vi "lire config gene.vi"(2 "error in":errorcluster, 3 "refnum":T1) -> (0 "error out":errorcluster, 1 "refnum out":T1)   [LabVIEW 2022 SP3]
uses:
  <vilib>/Utility/config.llb/Config Data RefNum.ctl
  <vilib>/Utility/config.llb/Read Key (Path).vi
  Variables globales/Variable glob generale.vi
  <vilib>/Utility/config.llb/Read Key (String).vi
  Variables globales/Variable glob mails.vi
  <vilib>/Utility/config.llb/NI_LVConfig.lvlib
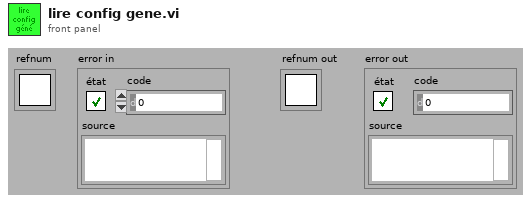
[diagram p1: front panel]
types:
  T1 = typedef "NI_LVConfig.lvlib/Config Data RefNum.ctl" = refnum<k1>
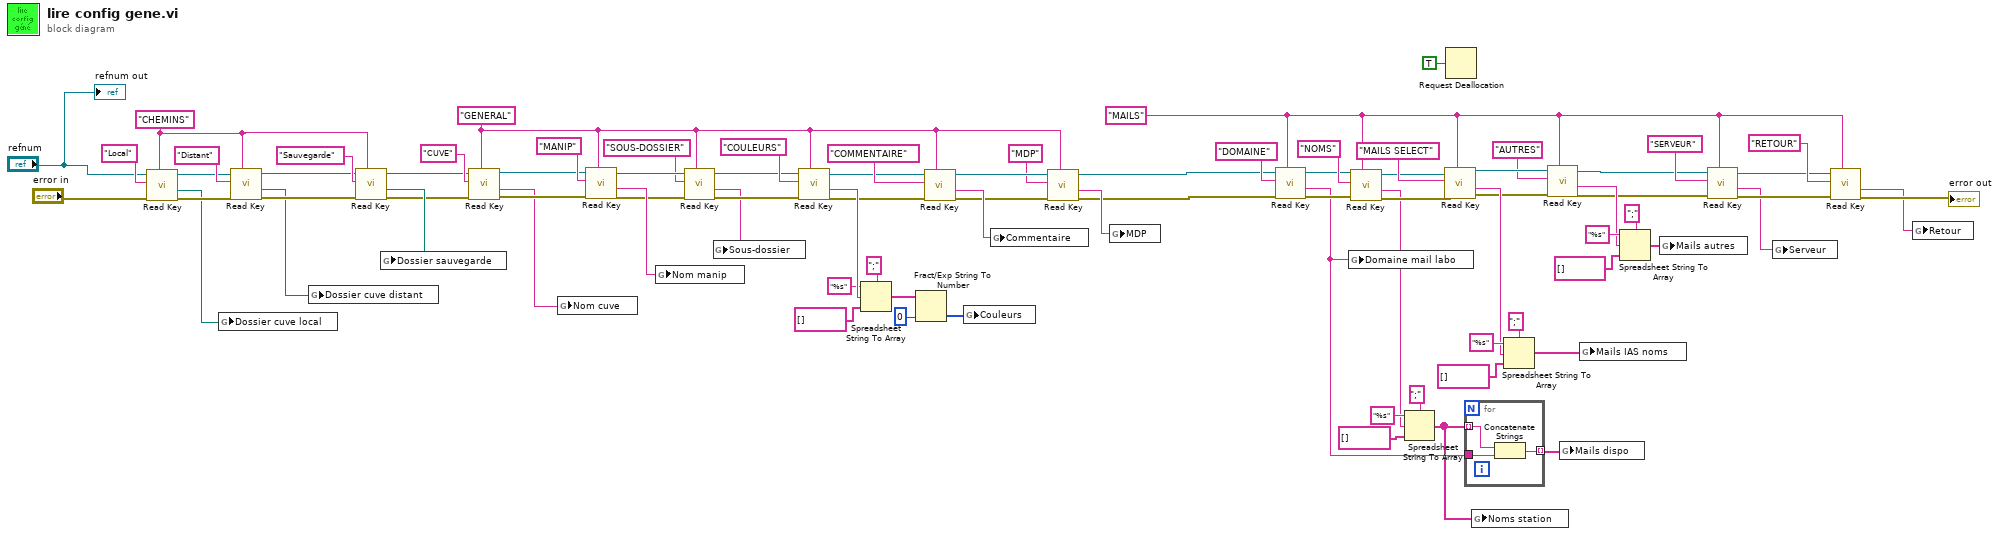
[diagram p0: block diagram]
diagram:
  w19 = "MAILS" ("section")
  w59 = "CHEMINS" ("section")
  w8 = "GENERAL" ("section")
  n1 = call-poly <vilib>:"Read Key.vi"("section"=w59, "error in (no error)"="error in", "key"="Local", "refnum"="refnum") -> ("error out"=w77:errorcluster, "value"=w42:path, "refnum out"=w76:T1)  [unwired: 4 in, 1 out]
  n2 = global write "Variable glob generale.vi" "Dossier cuve local"(w42) -> ()
  n3 = call-poly <vilib>:"Read Key.vi"("section"=w59, "error in (no error)"=w77, "key"="Distant", "refnum"=w76) -> ("error out"=w56:errorcluster, "value"=w43:path, "refnum out"=w57:T1)  [unwired: 4 in, 1 out]
  n4 = global write "Variable glob generale.vi" "Dossier cuve distant"(w43) -> ()
  n5 = call-poly <vilib>:"Read Key.vi"("section"=w59, "error in (no error)"=w56, "key"="Sauvegarde", "refnum"=w57) -> ("error out"=w45:errorcluster, "value"=w60:path, "refnum out"=w46:T1)  [unwired: 4 in, 1 out]
  n6 = global write "Variable glob generale.vi" "Dossier sauvegarde"(w60) -> ()
  n7 = call-poly <vilib>:"Read Key.vi"("section"=w8, "error in (no error)"=w45, "key"="CUVE", "refnum"=w46) -> ("error out"=w47:errorcluster, "value"=w41:string, "refnum out"=w48:T1)  [unwired: 4 in, 1 out]
  n8 = global write "Variable glob generale.vi" "Nom cuve"(w41) -> ()
  n9 = call-poly <vilib>:"Read Key.vi"("section"=w8, "error in (no error)"=w47, "key"="MANIP", "refnum"=w48) -> ("error out"=w53:errorcluster, "value"=w55:string, "refnum out"=w54:T1)  [unwired: 4 in, 1 out]
  n10 = global write "Variable glob generale.vi" "Nom manip"(w55) -> ()
  n11 = call-poly <vilib>:"Read Key.vi"("section"=w8, "error in (no error)"=w53, "key"="SOUS-DOSSIER", "refnum"=w54) -> ("error out"=w51:errorcluster, "value"=w49:string, "refnum out"=w52:T1)  [unwired: 4 in, 1 out]
  n12 = global write "Variable glob generale.vi" "Sous-dossier"(w49) -> ()
  n13 = call-poly <vilib>:"Read Key.vi"("section"=w8, "error in (no error)"=w51, "key"="COULEURS", "refnum"=w52) -> ("error out"=w37:errorcluster, "value"=w84:string, "refnum out"=w36:T1)  [unwired: 4 in, 1 out]
  n14 = Spreadsheet String To Array(delimiter (Tab)=";" ("séparateur (Tabulation)"), format string="%s" ("chaîne de format"), spreadsheet string=w84, array type (2D Dbl)=string[] [] ("type de tableau (2D de dbl)")) -> (array=w11:string[])
  n15 = Fract/Exp String To Number(string=w11, default (0 dbl)=u32 0 ("valeur par défaut (0 DBL)")) -> (number=w10:u32[])  [unwired: 2 in, 1 out]
  n16 = call-poly <vilib>:"Read Key.vi"("section"=w8, "error in (no error)"=w37, "key"="COMMENTAIRE", "refnum"=w36) -> ("error out"=w6:errorcluster, "value"=w38:string, "refnum out"=w7:T1)  [unwired: 4 in, 1 out]
  n17 = global write "Variable glob generale.vi" "Couleurs"(w10) -> ()
  n18 = global write "Variable glob generale.vi" "Commentaire"(w38) -> ()
  n19 = call-poly <vilib>:"Read Key.vi"("section"=w8, "error in (no error)"=w6, "key"="MDP", "refnum"=w7) -> ("error out"=w2:errorcluster, "value"=w4:string, "refnum out"=w3:T1)  [unwired: 4 in, 1 out]
  n20 = global write "Variable glob generale.vi" "MDP"(w4) -> ()
  n21 = call-poly <vilib>:"Read Key.vi"("section"=w19, "error in (no error)"=w2, "key"="DOMAINE", "refnum"=w3) -> ("error out"=w25:errorcluster, "value"=w17:string, "refnum out"=w26:T1)  [unwired: 4 in, 1 out]
  n22 = global write "Variable glob mails.vi" "Domaine mail labo"(w17) -> ()
  n23 = call-poly <vilib>:"Read Key.vi"("section"=w19, "error in (no error)"=w25, "key"="NOMS", "refnum"=w26) -> ("error out"=w23:errorcluster, "value"=w18:string, "refnum out"=w24:T1)  [unwired: 4 in, 1 out]
  n24 = Spreadsheet String To Array(delimiter (Tab)=";" ("séparateur (Tabulation)"), format string="%s" ("chaîne de format"), spreadsheet string=w18, array type (2D Dbl)=string[] [] ("type de tableau (2D de dbl)")) -> (array=w14:string[])
  n25 = call-poly <vilib>:"Read Key.vi"("section"=w19, "error in (no error)"=w23, "key"="MAILS SELECT", "refnum"=w24) -> ("error out"=w67:errorcluster, "value"=w69:string, "refnum out"=w66:T1)  [unwired: 4 in, 1 out]
  n26 = Request Deallocation(TRUE ("flag")) -> ()
  n27 = for {
    tunnel: w14 -> [w86] mode=indexing
    tunnel: w17 -> [w87]
    tunnel: [w85] -> w1 mode=indexing
    n28 = Concatenate Strings(w86, w87) -> (w85:string)
  }
  n29 = global write "Variable glob mails.vi" "Noms station"(w14) -> ()
  n30 = Spreadsheet String To Array(delimiter (Tab)=";" ("séparateur (Tabulation)"), format string="%s" ("chaîne de format"), spreadsheet string=w69, array type (2D Dbl)=string[] [] ("type de tableau (2D de dbl)")) -> (array=w16:string[])
  n31 = call-poly <vilib>:"Read Key.vi"("section"=w19, "error in (no error)"=w67, "key"="AUTRES", "refnum"=w66) -> ("error out"=w29:errorcluster, "value"=w61:string, "refnum out"=w30:T1)  [unwired: 4 in, 1 out]
  n32 = global write "Variable glob mails.vi" "Mails dispo"(w1) -> ()
  n33 = global write "Variable glob mails.vi" "Mails IAS noms"(w16) -> ()
  n34 = Spreadsheet String To Array(delimiter (Tab)=";" ("séparateur (Tabulation)"), format string="%s" ("chaîne de format"), spreadsheet string=w61, array type (2D Dbl)=string[] [] ("type de tableau (2D de dbl)")) -> (array=w15:string[])
  n35 = global write "Variable glob mails.vi" "Mails autres"(w15) -> ()
  n36 = call-poly <vilib>:"Read Key.vi"("section"=w19, "error in (no error)"=w29, "key"="SERVEUR", "refnum"=w30) -> ("error out"=w32:errorcluster, "value"=w12:string, "refnum out"=w33:T1)  [unwired: 4 in, 1 out]
  n37 = global write "Variable glob mails.vi" "Serveur"(w12) -> ()
  n38 = call-poly <vilib>:"Read Key.vi"("section"=w19, "error in (no error)"=w32, "key"="RETOUR", "refnum"=w33) -> ("error out"=→"error out":errorcluster, "value"=w13:string)  [unwired: 4 in, 2 out]
  n39 = global write "Variable glob mails.vi" "Retour"(w13) -> ()
  "refnum out" <- "refnum"
